vi "AlliGator Phasor Plot Panel.vi"() -> ()   [LabVIEW 2021, in "AlliGator Phasor Plot.lvlib"]
uses:
  AlliGator Phasor Plot.lvlib
  Phasor/Phasor (g, s).ctl
  Phasor/Phasor (m, phi).ctl
  AlliGator Phasor Plot Ctrl Refnums.ctl
  Globals, Variables, Constants/AlliGator Refnums List.ctl
  Utilities/Read-Write.ctl
  Settings/AlliGator Settings List.ctl
  Globals, Variables, Constants/AlliGator Variables List.ctl
  Palette/Image Palette Information.ctl
  Image/Image Display Palette Type.ctl
  Image/Image Display Event.ctl
  Image/Image Control Refnum.ctl
  <vilib>/Utility/miscctls.llb/LVPoint32TypeDef.ctl
  Action Engine/AlliGator Q Element.ctl
  Action Engine/AlliGator Q Event.ctl
  Image/Image Display User Event Data.ctl
  GUI/AlliGator Image Mouse Up Event Data.ctl
  Image/Image ROI Descriptor.ctl
  Image/Image Contour Definition.ctl
  Image/Image Contour ID.ctl
  Image/Image ROI Type.ctl
  Variant/Variant to Data/Variant to Boolean.vi
  Variant/Variant to Data/Variant to [String].vi
  Settings/AlliGator Settings+.lvlib
  Variant/Variant to Data/Variant to Data.lvlib
  Notebook/Notebook.lvlib
  Action Engine/AlliGator Action Engine.lvlib
  GUI/GUI.lvlib
  GUI/AlliGator GUI.lvlib
  Error/Error.lvlib
  Image/Image.lvlib
  Palette/Palette.lvlib
  Globals, Variables, Constants/AlliGator Globals, Variables & Constants.lvlib
  Python Plugins API/AlliGator Python Plugins.lvlib
  Phasor Graph/AlliGator Phasor Graph.lvlib
  Utilities/Utilities.lvlib
  Phasor/Phasor.lvlib
panel:
  out "True Phasor Plot Value":i32
  in  "Phasor ROI Decay":bool
  in  "Clear Phasor Overlay":bool
  in  "Highlight Phasor in Source Image":bool caption="Highlight Phasor ROI"
  in  "Image Overlay Color":u32(colorbox)=16777216
  in  "Overlay Mode":u16(ring)
  in  "Phasor Plot Active":bool
  in  "Pin Button":bool=TRUE
  in  "Phasor Plot ROI Color":u32(colorbox)=6618880
  in  "Refresh Phasor Plot":bool caption="Refresh Phsor Plot"
  out "Phasor Plot Image":T1(plugin-control)
  out "Phasor Plot Average Lifetime":dbl[unit]=nan caption="<tau>_a" format="%#_4e"
  out "Phasor Plot Phasor Ratio":dbl=nan caption="Amplitude Ratio (a1)" format="%#_4e"
  out "Phasor Plot Modulus Lifetime":dbl[unit]=nan caption="Modulus Lifetime" format="%#_4e"
  out "Phasor Plot Phase Lifetime":dbl[unit]=-9.431404035075279e-09 caption="Phase Lifetime" format="%#_4e"
  out "Phasor at cursor (m, phi)":T2={"m"=1.5330078000581284, "phi"=1.7786862539971595} caption="Phasor at Cursor (m, phi)" {"phi" format="%#_4e"; "m" format="%#_4e"}
  out "Phasor at cursor (g, s)":T3={"g"=-0.31640625, "s"=1.5} caption="Phasor at Cursor" {"s" format="%#.3e"; "g" format="%#_4e"}
  in  "Phasor Plot Color Scale":dbl(ramp)
  in  "Phasor Plot Display Range":cluster{u32, u32}(slide)={0, 100} scale=0.0..6578.0
  in  "Save Phasor Plot":bool
  out "Reference 2 Button":bool caption="Reference"
  out "Reference 1 Button":bool caption="Reference"
  in  "Phasor Plot Frequency":dbl[unit]=80000000.0 caption="Phasor Frequency"
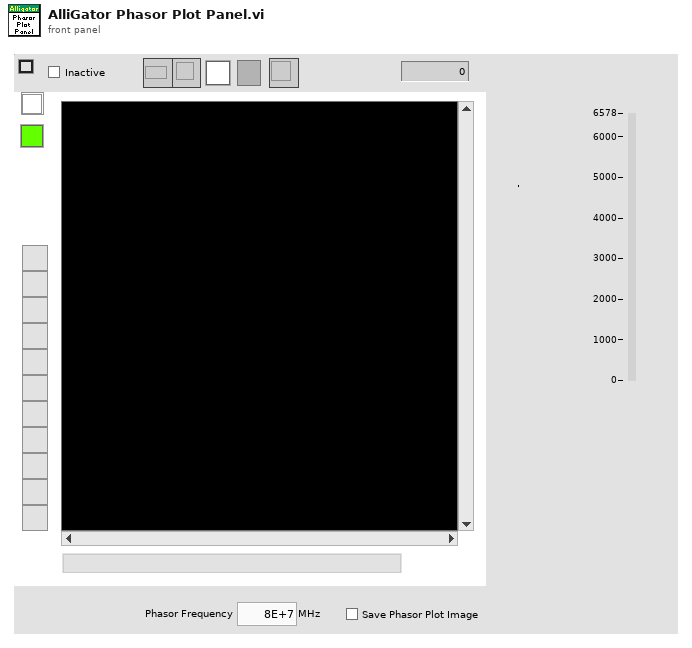
[diagram p1: front panel]
types:
  T1 = typedef "IMAQ Image.ctl" = refnum<image>
  T2 = typedef "Phasor.lvlib/Phasor (m, phi).ctl" = cluster{"m":dbl, "phi":dbl}
  T3 = typedef "Phasor.lvlib/Phasor (g, s).ctl" = cluster{"g":dbl, "s":dbl}
  T4 = typedef "Utilities.lvlib/Read-Write.ctl" = enum16{"Read", "Write"}
  T5 = typedef "AlliGator GUI.lvlib/AlliGator Refnums List.ctl" = enum16{"---------- AlliGator Control Refnums ----------", "AlliGator Tab Control Refnum", "Dataset Ctrl Refnums", "Image Histogram Ctrl Refnums", "Intensity Time Trace Ctrl Refnums", "Decay Graph Ctrl Refnums", "Decay Statistics Graph Ctrl Refnums", "Phasor Graph Ctrl Refnums", "Phasor Ratio Graph Ctrl Refnums", "Phasor Plot Ctrl Refnums", "Lifetime & Other Parameters Ctrl Refnums", "Decay Fit Parameter Map Ctrl Refnums", "Parameter Map Ctrl Refnums", "Other AlliGator Ctrl Refnums", "---------- AlliGator Menu Refnums ----------", "AlliGator Menu", "---------- IO Device ID ----------", "Mouse ID", "Keyboard ID"}
  T6 = typedef "AlliGator Phasor Plot.lvlib/AlliGator Phasor Plot Ctrl Refnums.ctl" = cluster{"Phasor Ratio":refnum<vi>, "Modulus Lifetime":refnum<vi>, "Phasor at cursor (m, phi)":refnum<vi>, "Phase Lifetime":refnum<vi>, "Phasor at cursor (g, s)":refnum<vi>, "Phasor Plor Average Lifetime":refnum<vi>, "Phasor Plot Active":refnum<vi>, "Save Phasor Plot":refnum<vi>, "Image Overlay Color":refnum<vi>, "Phasor Plot Color Scale":refnum<vi>, "Reference 1 Button":refnum<vi>, "Reference 2 Button":refnum<vi>, "True Phasor Plot Value":refnum<vi>, "Phasor Plot Display Range":refnum<vi>, "Phasor Plot Display":refnum<vi>, "Phasor Plot Frequency":refnum<vi>, "Overlay Mode":refnum<vi>}
  T7 = cluster{"Event Registration Refnum":refnum<event-registration>, "Phasor Plot Display Event":refnum<event-registration>, "Phasor Plote Display Range Event":refnum<event-registration>}
  T8 = typedef "AlliGator Settings+.lvlib/AlliGator Settings List.ctl" = enum16{"GUI:Visible Settings Tab", "GUI:Last Run Version", "Source Image:Use Image Histogram for Contrast", "Source Image:Low Count Pixels Rejection Options", "Source Image:High Count Pixels Rejection Options", "Source Image:Use Image Brightness", "Source Image:Blend Overlay with Image Background", "Source Image:Use Fixed ROI Diameter", "Source Image:ROI Diameter", "Source Image:ROI Center Color", "Source Image:Peak Threshold", "Source Image:Intensity Threshold", "Source Image:Image Binning Options", "Source Image:Image Smoothing Options", "Source Image:Image Histogram Active", "Source Image:Invert Binary Mask", "Source Image:Hot Pixel Removal", "Source Image:Overlay Analyzed ROI Center", "Source Image:Auto-Adjust Contrast", "Source Image:Histogram Lower Percentile", "Source Image:Histogram Upper Percentile", "Source Image:Lock ROI with Maps", "Source Image:Save Source Image", "Source Image:Scale Bar Options", "Source Image:Image Resolution (Pixel Size)", "Source Image:Flatfield Correction", "Source Image:Show Dead Left Columns Correction", "Source Image:Dead Left Columns Correction", "Source Image:Image Pre-Processing Operations Order", "Source Image:Overlay ROI Median", "Source Image:Median Overlay Color", "Data Information:Gate Width", "Data Information:Nanotime Gate Separation", "Data Information:Macrotime Gate Separation", "Data Information:Gate Step", "Data Information:# Gates", "Data Information:Gate Image Exposure", "Data Information:Gate Image Integration", "Data Information:Gates to Skip", "Data Information:Gates to Keep", "Data Information:Define Gates to", "Data Information:Channel Name", "Data Information:Available Channel Names", "Data Information:Channel Arithmetic", "Data Information:Background File Subtraction", "Data Information:Background File", "Data Information:Background Scaling Factor", "Data Information:Background Pile-up Correction", "Data Information:Background Pixel Well Capacity", "Data Information:Laser Period", "Data Information:SYNC Period", "Data Information:Pile-up Correction", "Data Information:Pixel Well Capacity", "Data Information:Dataset Scaling Factor", "Fluorescence Decay_Decay Pre-Processing:Reverse Gates", "Fluorescence Decay_Decay Pre-Processing:Verbose Decay Pre-Processing", "Fluorescence Decay_Decay Pre-Processing:Use Decay Pre-Processing", "Fluorescence Decay_Decay Pre-Processing:Background Subtraction", "Fluorescence Decay_Decay Pre-Processing:Background Definition Range", "Fluorescence Decay_Decay Pre-Processing:Baseline Subtraction Method", "Fluorescence Decay_Decay Pre-Processing:Decay Pre-Processing Operations Order", "Fluorescence Decay_Decay Pre-Processing:Smoothing Parameter", "Fluorescence Decay_Decay Pre-Processing:Shift Decay", "Fluorescence Decay_Decay Pre-Processing:Decay Shift Parameters", "Fluorescence Decay_Decay Pre-Processing:Fold Decay", "Fluorescence Decay_Decay Pre-Processing:# Folds", "Fluorescence Decay_Decay Pre-Processing:1-Normalize Decay", "Fluorescence Decay_Decay Pre-Processing:[0-1]-Normalize Decay", "Fluorescence Decay_Decay Pre-Processing:Smoothen Decay", "Fluorescence Decay_Decay Pre-Processing:Extrapolate Decay", "Fluorescence Decay_Decay Pre-Processing:Use Periodicity", "Fluorescence Decay_Decay Pre-Processing:Use Cursors", "Fluorescence Decay_Decay Pre-Processing:Tail Fraction", "Fluorescence Decay_Decay Pre-Processing:Head Fraction", "Fluorescence Decay_Decay Pre-Processing:Additional Points", "Fluorescence Decay_Decay Pre-Processing:Straighten Decay", "Fluorescence Decay_Decay Pre-Processing:Constant Background", "Fluorescence Decay_Decay Pre-Processing:Pixel-Normalize Decay", "Fluorescence Decay_Advanced Analysis:Extract IRF instead of Decay", "Fluorescence Decay_Advanced Analysis:IRF Extraction Options", "Fluorescence Decay_Advanced Analysis:IRF Optimization Options", "Fluorescence Decay_Advanced Analysis:Square Pulse Options", "Fluorescence Decay_Advanced Analysis:IRF Order", "Fluorescence Decay_Advanced Analysis:IRF Time Constants", "Fluorescence Decay_Advanced Analysis:Wavelet Analysis Options", "Fluorescence Decay_Advanced Analysis:Average Lifetime Options", "Fluorescence Decay_Fit Options:Fit Options", "Fluorescence Decay_Fit Options:Use Legacy Fitting Approach", "Fluorescence Decay_Fit Options:Use Data Information Laser Period", "Fluorescence Decay_Fit Parameters:Displayed Fit Parameters", "Fluorescence Decay_Fit Parameters:Fit Parameter Constraints", "Fluorescence Decay_Fit Parameters:Export Tabulated Results", "Fluorescence Decay_Fit Parameters:MLE Baseline Offset Type", "Fluorescence Decay_Fit Parameters:MLE Baseline Offset", "Fluorescence Decay_Fit Parameters:Guess Parameter Names", "Fluorescence Decay_Fit Parameters:Guess Parameter Values", "Fluorescence Decay_Fit Parameters:Guess Parameters Options", "Fluorescence Decay_Fit Parameters:Optimal Offset Selection Criterion", "Fluorescence Decay_Styles:Show Last Decay Only", "Fluorescence Decay_Styles:Decay Graph Color Array", "Fluorescence Decay:Decay Graph Active", "Fluorescence Decay Statistics:Min Peak Value", "Fluorescence Decay Statistics:Reject Low Decay Peak Pixels", "Fluorescence Decay Statistics:Reject High Decay Peak Pixels", "Fluorescence Decay Statistics:Max Peak Value", "Time Traces:Use File Timestamp", "Time Traces:Time Step", "Time Traces:Use Intensity Correction File", "Time Traces:Intensity Correction File", "Phasor Plot:Phasor Plot Smoothing Options", "Phasor Plot:Phasor Plot Size", "Phasor Plot:Phasor Plot Graphics Options", "Phasor Plot:Cumulative Phasor Plot", "Phasor Plot:Use Phasor Brightness", "Phasor Plot:Blend Overlay with Phasor Background", "Phasor Plot:Save Phasor Plot", "Phasor Plot:Show References", "Phasor Plot:Phasor Ratio Decay Range", "Phasor Plot:Exponential Fading", "Phasor Plot:Phasor Ratio Reference Colors", "Phasor Plot:Reference Radius", "Phasor Plot:Show Color Map Vertices", "Phasor Plot:Phasor Plot Active", "Phasor Plot:Phasor Ratio Color Map Type", "Phasor Plot:Phasor Ratio Color Map", "Phasor Plot:Phasor Ratio Display Range", "Phasor Plot:Selected Image ROI(s)", "Phasor Plot:All Image ROIs", "Phasor Plot:Selected Phasor Plot ROI(s)", "Phasor Plot:All Phasor Plot ROIs", "Phasor Plot:Phasor Ratio Color-Coded Quantity", "Phasor Plot:Store Phasor Harmonics", "Phasor Plot:Draw Reference Segment", "Phasor Plot:User-Defined Quantity", "Phasor Plot:Color Scale High Color", "Phasor Plot:Color Scale Low Color", "Phasor Plot:Intensity-weighted Phasor Plot", "Phasor Graph:Phasor Frequency", "Phasor Graph:Phasor Ratio Type", "Phasor Graph:Pixel-level Phasor Computation", "Phasor Graph:Save Phasor Graph", "Phasor Graph:Phasor Graph Active", "Phasor Graph:Phasor SDV Options", "Phasor Graph:Intensity-weighted Phasor Graph", "Phasor Graph:Define Shortest Lifetime as", "Phasor Calibration:Use Backup Calibration if needed", "Phasor Calibration:Backup Calibration Type", "Phasor Calibration:Calibration Type", "Phasor Calibration:Calibration Lifetime", "Phasor Calibration:Calibration Map Algorithm", "Single-Exponential Phasor Locus (SEPL):Gate Parameters", "Single-Exponential Phasor Locus (SEPL):User-defined Gate", "Single-Exponential Phasor Locus (SEPL):User-defined IRF", "Single-Exponential Phasor Locus (SEPL):Phasor Parameters", "Single-Exponential Phasor Locus (SEPL):Decay & IRF Parameters", "Single-Exponential Phasor Locus (SEPL):Display Parameters", "Lifetime Analysis:Decay Analysis Parameters", "Lifetime Analysis:Lifetime Map Active", "Plugins:Python Settings", "Miscellaneous:Verbose Mode", "Miscellaneous:Beep after Script", "Miscellaneous:Saved Image File Format", "Miscellaneous:Exported Gate Image Settings", "Miscellaneous:Include Loading in Timing", "Miscellaneous:Verbose Settings Mode", "Miscellaneous:Histogram Options", "Miscellaneous:Beep on Error", "Miscellaneous:# Logical Processors Used", "Miscellaneous:ROI Description Max Characters", "Miscellaneous:Verbose Error Mode", "Miscellaneous:Transparent Mask Color"}
  T9 = typedef "Palette.lvlib/Image Palette Information.ctl" = cluster{"Palette Name [# Colors,int?,inv?]":string, "Palette Type":T10, "Palette Colors":u32[], "Interpolate?":bool}
  T10 = typedef "Image.lvlib/Image Display Palette Type.ctl" = u32
  T11 = typedef "AlliGator Globals, Variables & Constants.lvlib/AlliGator Variables List.ctl" = enum16{"---- GUI ----", "GUI:Initialization Status", "GUI:State Indicators Refnum", "GUI:Original AlliGator Menu Items", "GUI:Current Action Loop State", "GUI:Script in progress", "GUI:Playback", "GUI:Loop Playback", "GUI:Search ROI Used", "GUI:Search ROI", "Image Histogram Max Legend Size", "Decay Graph Max Legend Size", "Intensity Graph Max Legend Size", "Decay Statistics Graph Max Legend Size", "Phasor Graph Max Legend Size", "Phasor Ratio Graph Max Legend Size", "Lifetime Graph Max Legend Size", "---- Files ----", "Files:Export Dataset Frames as Individual Files", "Files:Show Batch Export Help Balloons", "Files:Frames in Dataset", "Files:ptu File Frame Start Indices", "Files:Current Frame in Dataset", "Files:Current Frame Timestamp", "Files:Dataset Loaded", "Files:Dataset Metadata", "Files:Dataset Channel", "Files:Dataset Data Description", "Files:Background Dataset Metadata", "Files:Background Dataset Channel", "Files:Background Dataset Data Description", "Files:Background File Subtraction", "Files:Background File Path", "Files:Background File Pile-up Correction", "Files:Background File Pixel Well Capacity", "Files:Background File Scaling Factor", "Files:Current Dataset Load Settings", "Files:Dataset Path", "Files:ICCD-specific Information", "Files:Macrotime Gate Separation", "------ Python Plugins ------", "Python Plugins:Information", "Python Plugins:Python Session", "Python Plugins:Valid Python Session?", "---- Source Image ----", "Source Image:ROIs", "Source Image:Current ROI", "Source Image:ROI Event Refnum", "X_Source Image:Display Range", "X_Source Image:Palette Information", "X_Source Image:Type of Displayed Image", "X_Time Gate Slider", "Source Image:Palette List", "Source Image:Scale", "Source Image:ROI Overlay Color", "Source Image:Overlay to Erase", "Source Image:Is Displayed Image Accumulated", "Source Image:White Light Image Modified", "Source Image:Mask Image Modified", "---- Image Profile Window ----", "Image Profile:Window Event Refnum", "Image Profile:IntensityType", "Image Profile:Intensity Average Type", "Image Profile:Intensity-weighted SDV", "Image Profile:Box Profile Type", "Image Profile:Window Open", "Image Profile:Plotted Fit Parameter", "------ Phasor Graph -------", "Phasor Graph:Show Line", "---- Phasor Plot ---", "Phasor Plot:Parameters Changed", "Phasor Plot:FLI Dataset Modified since last Calculation", "Phasor Harmonics Data", "Selected Phasor Harmonics", "Phasor Harmonic Manager Event Refnum", "Phasor Plot:ROIs", "Phasor Plot:Current ROI", "Phasor Plot:ROI Event Refnum", "Phasor Plot:Image Reference Points", "Phasor Plot:Computed", "Phasor Plot:Palette Information", "Phasor Plot:Palette List", "Phasor Plot:Phasor Ratio Palette Information", "Phasor Plot:Phasor Ratio Palette List", "Phasor Plot:Image Scale", "Phasor Plot:Image Overlay to Erase", "Phasor Plot:Image Elements to Update", "Phasor Plot:Current Calculation Parameters", "Phasor Plot:Current Calibration Options", "Phasor Plot:Reset Cumulated Phasor Plot", "Phasor Plot:Reference 1", "Phasor Plot:Lifetime Reference 1", "Phasor Plot:Reference 1 Frequency", "Phasor Plot:Reference 2", "Phasor Plot:Lifetime Reference 2", "Phasor Plot:Reference 2 Frequency", "---- Decay Analysis ----", "Number of Selected Decays to Fit", "LS Fit Results", "LAR Fit Results", "BS Fit Results", "Last Decay Max - Min", "Best Fit Parameters", "Best Fit Parameter Names", "Actual Size X", "Actual Size Y", "Binning X", "Binning Y", "Actual # Gates", "Dataset Number", "Gates to...", "Gates Skipped", "Gates to keep", "Gate Step", "Gate Separation", "Reversed Gates", "Pile-up Correction", "Pixel Well Capacity", "Background Subtracted", "Background Subtraction Method", "Background Definition Range", "Background File (deprecated)", "Number of Dataset Accumulated", "Array of Accumulated Dataset Paths", "Do Averaged Datasets", "Destination File Path", "Process Plot Target", "Use 1/D as Phasor Frequency", "---- Decay Fit Parameter Map -----", "Decay Fit Parameter Map:Palette Information", "Decay Fit Parameter Map:Palette List", "Decay Fit Parameter Map:X Resolution", "Decay Fit Parameter Map:Y Resolution", "Decay Fit Parameter Map:Use Decay Fit Result Constraints", "Decay Fit Parameter Map:Decay Fit Result Constraints", "Decay Fit Parameter Map:Decay Fit Result Constraints Applied", "---- Parameter Map ----", "Parameter Map:Palette Information", "Parameter Map:Palette List", "------- Local Decay Window ---------", "Local Decay Graph Window:Event Refnum", "Local Decay Graph Window:Use normalized IRF for convolution", "----- Miscellaneous ----", "Misc:Skippable Dialog Windows Status"}
  T12 = enum16{"0", "1", "2", "3", "4", "5", "6", "7", "8", "9", "A", "B", "C", "D", "E", "F", "G", "H", "I", "J", "K", "L", "M", "N", "O", "P", "Q", "R", "S", "T", "U", "V", "W", "X", "Y", "Z", "F1", "F2", "F3", "F4", "F5", "F6", "F7", "F8", "F9", "F10", "F11", "F12", "F13", "F14", "F15", "ADD", "BACK", "BACKSLASH", "CAPITAL", "COMMA", "DECIMAL", "DELETE", "DIVIDE", "DOWN", "END", "EQUALS", "ESCAPE", "GRAVE (`)", "HOME", "INSERT", "LBRACKET", "LCONTROL", "LEFT", "L ALT", "LSHIFT", "LWIN", "MINUS", "MULTIPLY", "NEXT", "NUMLOCK", "NUMPAD_0", "NUMPAD_1", "NUMPAD_2", "NUMPAD_3", "NUMPAD_4", "NUMPAD_5", "NUMPAD_6", "NUMPAD_7", "NUMPAD_8", "NUMPAD_9", "PAUSE", "PERIOD", "PRIOR (PG UP)", "RBRACKET", "RCONTROL", "RETURN", "RIGHT", "R ALT", "RSHIFT", "RWIN", "SCROLL", "SEMICOLON", "SLASH", "SPACE", "SUBTRACT", "TAB", "UP", "ENTER (num pad)", "' (quote)"}
  T13 = typedef "Image.lvlib/Image Display Event.ctl" = cluster{"Item Tag":string, "Image Control Refnum":T14, "Coords":T15, "Item Path":string}
  T14 = typedef "Image.lvlib/Image Control Refnum.ctl" = refnum<vi>
  T15 = typedef "LVPoint32TypeDef.ctl" = cluster{"Horizontal":i32, "Vertical":i32}
  T16 = typedef "AlliGator Action Engine.lvlib/AlliGator Q Element.ctl" = cluster{"AlliGator Q Event":T17, "Data":variant}
  T17 = typedef "AlliGator Action Engine.lvlib/AlliGator Q Event.ctl" = enum16{"---- Files ----", "Files:Set Batch Export Files To Save", "Files:Set Dataset Loading & Pre-processing Options", "Files:Check #Frames in Dataset", "Files:Increment Frame Index", "Files:Open Mask Image", "Files:Open White Light Image", "Files:Open Single Dataset", "Files:New Folder of Folders Selected", "Files:Load File (all Types)_Scriptable", "Files:Move Flattened Series to Folders Series", "Files:Select Folder", "Files:Load FLI Dataset", "Files:Load Swiss SPAD 1 Dataset", "Files:Load Swiss SPAD 2 Dataset", "Files:Load .sdt FLI Dataset", "Files:Load .ptu FLI Dataset", "Files:Load .bin FLI Dataset", "Files:Load Single Gate Image Folder", "Files:Load I/m/phi Dataset (deprecated)", "Files:Load Single Image", "Files:Subtract Background File", "Files:Export FLI Dataset", "Files:Load HDF5 FLI Dataset", "Files:Set Destination File Path", "Files:Save Mask Image", "Files:Batch Conversion", "Files:New Folder Selected", "Files:Close FLI Dataset", "Files:Close FLI Dataset Series", "Files:Close White Light Image", "Files:Close Mask Image", "---- FLI Dataset ----", "FLI Dataset:Channel Arithmetic", "FLI Dataset:Export Average Lifetime Map as ASCII", "FLI Dataset:Export User-Defined Quantity Map as ASCII", "FLI Dataset:Python Function FLI Dataset Event", "FLI Dataset:ROI Analysis", "FLI Dataset:Tilted Logistic Square Gated IRF Characteristics Map", "FLI Dataset:Logistic Square Gated IRF Characteristics Map", "FLI Dataset:Square Gated IRF Characteristics Map", "FLI Dataset:Multi-ROI Single-Pixel Phasor Analysis", "FLI Dataset:Multi-ROI Single-Pixel NLSF Analysis", "FLI Dataset:All ROIs IRF Extraction", "FLI Dataset:All ROIs Decay Fit Non-Interactive (Fast + Individual IRF)", "FLI Dataset:All ROIs Phasor Analysis", "FLI Dataset:All ROIs Decay Fit", "FLI Dataset:Fluorescence Decay Statistics", "FLI Dataset:Update Decay Statistics Graph", "FLI Dataset:Get Decay from ROI", "FLI Dataset:All ROIs Average Lifetimes", "FLI Dataset:Save/Load Local IRFs", "FLI Dataset:Clear Local IRFs", "FLI Dataset:Phasor Calibration Maps (# Gates Series) Script", "FLI Dataset:Calibrated Phasor Map Series", "---- FLI Dataset Series ----", "FLI Dataset Series:Sum All Datasets in Series", "FLI Dataset Series:Add Dataset to Accumulated Dataset", "FLI Dataset Series:Display Accumulated Dataset", "FLI Dataset Series:Clear Dataset Series Sum", "FLI Dataset Series:Time-Series Analysis (NLSF)", "FLI Dataset Series:Time-Series Analysis (Phasor)", "---- Image ----", "Image:Update Image Profile Plots", "Image:Image Histogram Cursor Move", "Image:Image Histogram", "Image:Image Contrast", "Image:Set Image Histogram Cursor Move Flag", "Image:Clear Image Overlay", "Image:Use ROI as Search Area", "Image:Set ROI Diameter", "Image:Save Image Data as TIFF", "Image:Save Displayed Image with Overlay", "Image:Save Image Overlay Only", "Image:Save Image as Hot Pixel Mask", "Image:Change Source Image Color Palette", "Image:Copy Image to Clipboard", "Image:Source Image ROI Selection", "Image:Delete All ROIs", "Image:Delete All Unselected ROIs", "Image:Delete ROI", "Image:Merge All ROIs", "Image:Store ROI", "Image:Source Image ROI Storage", "Image:Export ROI Description to Notebook", "Image:Save ROI", "Image:Load ROI", "Image:Paste ROI Definition", "Image:Clear ROI", "Image:Identify ROIs in Mask Image", "Image:Create Complementary ROI", "Image:Create Contour ROI", "Image:Create ROI(s) from Pixels with Peak above Min_Scriptable", "Image:Create ROI(s) from Pixels with Intensity above Min_Scriptable", "Image:Compute ROI Statistics", "Image:Delete ROI(s) based on ROI Characteristics", "Image:Create ROI Grid", "Image:ROI to Individual Pixel ROIs", "Image:Python Function Source Image Event", "Image:Show Phasor Calibration Map ROI Centers", "Image:Convert ROI to Mask Image", "Image:Mouse Move", "Image:Mouse Up", "Image:Set Source Image Mouse Move Flag", "Image:Add Scale Bar Overlay", "Image:Delete Existing ROIs Option", "Image:Overlay ROI Median", "Image:Check Current ROI", "Image:Update True Pixel Value", "Image:Use ROI", "---- Decay ----", "Decay:Clear IRF/Reference Plot", "Decay:Add Decay to Graph", "Decay:Smoothen Plot", "Decay:Smoothen Plot Tail", "Decay:Average Selected Plots", "Decay:Extract IRF", "Decay:Optimal IRF Extraction", "Decay:Threshold IRF", "Decay:Fit to Model IRF", "Decay:Fit IRF to Square Gate", "Decay:Fit IRF to Logistic Square Gate", "Decay:Fit IRF to Tilted Logistic Square Gate", "Decay:Create Bounding Cursors Set", "Decay:Export Bounding Cursors Definition to Notebook", "Decay:Denoise Plot", "Decay:Compute Cumulative Function", "Decay:Use as Reference Decay", "Decay:Show Reference Decay/IRF", "Decay:Extrapolate Decay", "Decay:Create Head & Tail Bounding Cursors", "Decay:Store Cursor-defined Head & Tail Fractions", "Decay:Rebin Plot", "Decay:1-Normalize Decay", "Decay:[0-1]-Normalize Plot", "Decay:Straighten Decay", "Decay:Shift Decay", "Decay:Fold Decay", "Decay:Fit Decay", "Decay:Global Fit of Selected Decays", "Decay:Post Global Fit Script", "Decay:Add Global Fit Parameters to Graph", "Decay:Add Decay Parameter(s) to Plot (Graph)", "Decay:Export Decay to Phasor Graph", "Decay:Compute Average Lifetime", "Decay:Plot Convolution", "Decay:Graph Tip Strip Update", "---- Decay Statistics ----", "Decay Statistics:Tip Strip Update", "---- Intensity Time Trace ----", "Intensity Time Trace:Use File Timestamp", "Intensity Time Trace:Load Intensity Corrections File", "Intensity Time Trace:Clear Intensity Corrections File", "Intensity Time Trace:Tip Strip Update", "---- Phasor Plot ----", "Phasor Plot:Build Phasor Plot", "Phasor Plot:Change Phasor Plot Color Palette", "Phasor Plot:Adjust Phasor Plot Display Range", "Phasor Plot:Highlight Image ROI in Phasor Plot", "Phasor Plot:Save Phasor Plot Image with Overlay", "Phasor Plot:Export Complex Phasor Map", "Phasor Plot:Export Phasor Ratio Map", "Phasor Plot:Export Average Lifetime Map", "Phasor Plot:Compute Phase Lifetime Histogram", "Phasor Plot:Compute Phasor Ratio Histogram", "Phasor Plot:Compute Phase Lifetime vs Intensity Scatter Plot", "Phasor Plot:Weber 2-Component Decomposition", "Phasor Plot:Update Phasor Color Map Vertices", "Phasor Plot:Clear Phasor Overlay", "Phasor Plot:Use Segment Extremities as References", "Phasor Plot:Use UC/Segment Intersections as References", "Phasor Plot:Use UC/Principal Axis Intersections as References", "Phasor Plot:Use UC/Linear Fit Intersections as References", "Phasor Plot:Update Phasor Plot Reference", "Phasor Plot:Show Local Phasor Info in Phasor Plot", "Phasor Plot:Update Phasor Plot State", "Phasor Plot:Phasor Plot ROI Storage", "Phasor Plot:Phasor Plot ROI Selection", "Phasor Plot:Python Function Phasor Plot Event", "Phasor Plot:Overlay Phasor ROI, Ratio or Map in Source Image", "Phasor Plot:Compute Decay of Selected Phasors", "Phasor Plot:Phasor at Image Pixel", "Phasor Plot:Mouse Move", "Phasor Plot:Mouse Up", "Phasor Plot:Display Range Mouse Move", "Phasor Plot:Set Mouse Move Flag", "Phasor Plot:Update True Phasor Plot Value", "---- Phasor Graph ----", "Phasor Graph:Get Phasor Value", "Phasor Graph:Create New Phasor Plot Dialog", "Phasor Graph:Update Last Phasor Value", "Phasor Graph:Update Phasor (m, phi)", "Phasor Graph:Remove Single Phasor from Plot", "Phasor Graph:Add Single Phasor to Plot", "Phasor Graph:Remove Phasor Plot", "Phasor Graph:Remove Selected Phasor Plots", "Phasor Graph:Clear Phasor Data", "Phasor Graph:Clear Phasor Graph", "Phasor Graph:Cursor Move", "Phasor Graph:Draw Cursor Connecting Line", "Phasor Graph:Clear Cursor Connecting Line", "Phasor Graph:Find UC Intersection", "Phasor Graph:Use UC/Cursor-Defined Line Intersections", "Phasor Graph:Use Selected Plots Fitted Line/UC Intersections", "Phasor Graph:Use Selected Plots Principal Axis/UC Intersections", "Phasor Graph:Show Single Phasor", "Phasor Graph:Save Single Phasor Plot", "Phasor Graph:Save All Phasor Plots", "Phasor Graph:Load Phasor Plot(s)", "Phasor Graph:Phasor Multiplication", "Phasor Graph:Compute Average Phasor", "Phasor Graph:Compute Multiple Average Phasors (Selected Plots)", "Phasor Graph:Export Single Phasor Plot Phase Lifetimes", "Phasor Graph:Parameter 2 vs Parameter 1 Scatter Plot", "Phasor Graph:Use Cursor n Location", "Phasor Graph:Set Reference n to Current Phase Lifetime Value", "Phasor Graph:Set Reference n to Lifetime Value", "Phasor Graph:Set Cursor n Location", "Phasor Graph:Save Phasor Graph Image", "Phasor Graph:Update SEPL Plot", "Phasor Graph:Export Single Phasor Plot Data", "Phasor Graph:Export Selected Phasor Plots Data", "Phasor Graph:Python Function Phasor Graph Event", "Phasor Graph:Tip Strip Update", "---- Calibration ----", "Calibration:Set Calibration Type", "Calibration:Load/Save Phasor Calibration", "Calibration:Load/Save Phasor Calibration Series", "Calibration:Load/Save Phasor Calibration Map", "Calibration:Use as Calibration", "Calibration:Compute Optimal Calibration from Phasor References", "Calibration:Clear Phasor Calibration", "Calibration:Single Phasor Calibration Information", "Calibration:Use as Calibration Series", "Calibration:Use as Calibration Map", "Calibration:Clear Calibration Series", "Calibration:Phasor Calibration Series Information", "Calibration:Clear Calibration Map", "Calibration:Phasor Calibration Map Information", "Calibration:Apply Phasor Calibration", "Calibration:Update Single Plot Calibration", "Calibration:Update Multiple Plots Calibration", "Calibration:Clear Single Plot Calibration", "Calibration:Clear All Plots Calibrations", "Calibration:Clear Plot(s) Calibration(s)?", "---- Phasor Ratio ----", "Phasor Ratio:Clear Reference n", "Phasor Ratio:Toggle Selected Plot(s)  Lock to Reference 1", "Phasor Ratio:Use as Reference n", "Phasor Ratio:Send Reference n to Notebook", "Phasor Ratio:Toggle Selected Plot(s)  Lock to Reference 2", "Phasor Ratio:Compute Phasor Ratio at Mouse Location", "Phasor Ratio:Compute Phasor Plot's Average Phasor Ratio", "Phasor Ratio:Compute Time-Series Phasor Ratios", "Phasor Ratio:Fit Line to Phasor Ratio Plot", "Phasor Ratio:Save References", "Phasor Ratio:Load References", "Phasor Ratio:Update Phasor Reference 1", "Phasor Ratio:Update Phasor Reference 2", "Phasor Ratio:Move Cursor n to Reference n", "Phasor Ratio:Use as Phasor Reference 1 Lifetime", "Phasor Ratio:Use as Phasor Reference 2 Lifetime", "Phasor Ratio:Export Phasor Ratio Map as ASCII", "Phasor Ratio:Tip Strip Update", "---- Lifetime & Other Parameters Graph ----", "Lifetime:Compute Sliced Mean, SDV and CV Plots", "Lifetime:Plot Decay Shifts", "Lifetime:Plot Histogram", "---- Decay Fit Parameter Map ----", "Decay Fit Parameter Map:Export ROI NLSF Data as ASCII", "Decay Fit Parameter Map:Set Decay Fit Parameter Map Selection", "Decay Fit Parameter Map:Build Decay Fit Parameter Map", "Decay Fit Parameter Map:Change Decay Fit Parameter Map Color Palette", "Decay Fit Parameter Map:Export Decay Fit Parameter Map Data as ASCII", "Decay Fit Parameter Map:Export All Decay Fit Parameter Maps Data as ASCII", "Decay Fit Parameter Map:Selected Parameter Scatterplot", "Decay Fit Parameter Map:Parameter 2 vs Parameter 1 Scatterplot", "Decay Fit Parameter Map:Save Decay Fit Parameter Map Image", "Decay Fit Parameter Map:Save-Load IRFs & Fit Data", "Decay Fit Parameter Map:Update Local Decay Plots", "Decay Fit Parameter Map:Python Function Decay Fit Parameters Map Event", "Decay Fit Parameter Map:Overlay Decay Fit Parameter Map in Source Image", "Decay Fit Parameter Map:Selected Parameter vs Intensity Scatterplot", "Decay Fit Parameter Map:Mouse Up", "Decay Fit Parameter Map:Mouse Move", "Decay Fit Parameter Map:Display Range Mouse Move", "Decay Fit Parameter Map:Change Map Resolution", "Decay Fit Parameter Map:Variance Significance Maps", "Decay Fit Parameter Map:Fit Result Constraints Window", "Decay Fit Parameter Map:Use ROI", "---- Parameter Map ----", "Parameter Map:Export ROI Parameters Data as ASCII", "Parameter Map:Add Parameter Map Set", "Parameter Map:Delete Parameter Map Set", "Parameter Map:Update Parameter List", "Parameter Map:Build Parameter Map", "Parameter Map:Change Parameter Map Color Palette", "Parameter Map:Export Parameter Map Data as ASCII", "Parameter Map:Export All Parameter Maps Data as ASCII", "Parameter Map:Selected Parameter Scatterplot", "Parameter Map:Parameter 2 vs Parameter 1 Scatterplot", "Parameter Map:Selected Parameter vs Intensity Scatterplot", "Parameter Map:Save Parameter Map Image", "Parameter Map:Save-Load IRFs & Parameter Maps (TODO)", "Parameter Map:Set Parameter Map Selection", "Parameter Map:Python Function Parameter Map Event", "Parameter Map:Overlay Parameter Map in Source Image", "Parameter Map:Update Local Decay Plots", "Parameter Map:Mouse Up", "Parameter Map:Mouse Move", "Parameter Map:Display Range Mouse Move", "Parameter Map:Use ROI", "---- Generic Graph ----", "Generic Graph:Generic XY Graph Event", "Generic Graph:Python Function XY Graph Event", "Generic Graph:New Plot", "Generic Graph:Save Plot", "Generic Graph:XY Plot Histogram", "Generic Graph:Set XY Graph Plot Name", "Generic Graph:Set Last Cursor Style", "Generic Graph:Tip Strip Update", "---- GUI ----", "GUI:Start Script", "GUI:Type of Displayed Image Changed", "GUI:Gate Image Slide Changed", "GUI:Show Busy Icon", "GUI:Show Busy Icon & Abort Button", "GUI:Hide Busy Icon", "GUI:Hide Busy Icon & Abort Button", "GUI:Abort", "GUI:End Script", "GUI:Start Timing", "GUI:End Timing", "GUI:Set State Indicator", "GUI:Send Parameters JSON Strings to Clipboard", "GUI:Set Gate Step", "GUI:Idle", "GUI:Initialization", "GUI:Quit", "GUI:Increment Dataset Index", "GUI:Set Dataset Index to -1", "GUI:Time Series Slider Moved", "GUI:Time Series Slider Changed", "GUI:Toggle Playback or Loop", "GUI:Playback Script", "GUI:Set Phasor Frequency", "GUI:Open Window", "GUI:Start Test Script", "GUI:End Test Script", "GUI:Set Verbose Mode", "GUI:Set Verbose Settings Mode", "GUI:Initialize Python Session", "DEBUG"}
  T18 = typedef "Image.lvlib/Image Display User Event Data.ctl" = cluster{"Image Control Refnum":T14, "Coords":T15, "button info":cluster{"button 1":bool, "button 2":bool, "button 3":bool, "button 4":bool}, "keys pressed":enum16{"0", "1", "2", "3", "4", "5", "6", "7", "8", "9", "A", "B", "C", "D", "E", "F", "G", "H", "I", "J", "K", "L", "M", "N", "O", "P", "Q", "R", "S", "T", "U", "V", "W", "X", "Y", "Z", "F1", "F2", "F3", "F4", "F5", "F6", "F7", "F8", "F9", "F10", "F11", "F12", "F13", "F14", "F15", "ADD", "BACK", "BACKSLASH", "CAPITAL", "COMMA", "DECIMAL", "DELETE", "DIVIDE", "DOWN", "END", "EQUALS", "ESCAPE", "GRAVE (`)", "HOME", "INSERT", "LBRACKET", "LCONTROL", "LEFT", "L ALT", "LSHIFT", "LWIN", "MINUS", "MULTIPLY", "NEXT", "NUMLOCK", "NUMPAD_0", "NUMPAD_1", "NUMPAD_2", "NUMPAD_3", "NUMPAD_4", "NUMPAD_5", "NUMPAD_6", "NUMPAD_7", "NUMPAD_8", "NUMPAD_9", "PAUSE", "PERIOD", "PRIOR (PG UP)", "RBRACKET", "RCONTROL", "RETURN", "RIGHT", "R ALT", "RSHIFT", "RWIN", "SCROLL", "SEMICOLON", "SLASH", "SPACE", "SUBTRACT", "TAB", "UP", "ENTER (num pad)", "' (quote)"}[]}
  T19 = typedef "AlliGator GUI.lvlib/AlliGator Image Mouse Up Event Data.ctl" = cluster{"Current ROI Tool":u32, "ROI Descriptor":T20, "Shift":bool, "Alt":bool, "Image Display Refnum":T14}
  T20 = typedef "Image.lvlib/Image ROI Descriptor.ctl" = cluster{"Global Rectangle":i32[], "Contours":T21[]}
  T21 = typedef "Image.lvlib/Image Contour Definition.ctl" = cluster{"Contour Type":T22, "ROI Type":T23, "Points":i32[]}
  T22 = typedef "Image.lvlib/Image Contour ID.ctl" = enum32{"External", "Internal"}
  T23 = typedef "Image.lvlib/Image ROI Type.ctl" = enum16{"No Selection", "Point", "Line", "Rectangle", "Oval", "Polygon", "Freehand Region", "Annulus", "Unused2", "Unused3", "Broken Line", "Freehand Line", "Rotated Rectangle"}
  T24 = enum16{"0", "1", "2", "3", "4", "5", "6", "7", "8", "9", "A", "B", "C", "D", "E", "F", "G", "H", "I", "J", "K", "L", "M", "N", "O", "P", "Q", "R", "S", "T", "U", "V", "W", "X", "Y", "Z", "F1", "F2", "F3", "F4", "F5", "F6", "F7", "F8", "F9", "F10", "F11", "F12", "F13", "F14", "F15", "ADD", "BACK", "BACKSLASH", "CAPITAL", "COMMA", "DECIMAL", "DELETE", "DIVIDE", "DOWN", "END", "EQUALS", "ESCAPE", "GRAVE (`)", "HOME", "INSERT", "LBRACKET", "LCONTROL", "LEFT", "L ALT", "LSHIFT", "LWIN", "MINUS", "MULTIPLY", "NEXT", "NUMLOCK", "NUMPAD_0", "NUMPAD_1", "NUMPAD_2", "NUMPAD_3", "NUMPAD_4", "NUMPAD_5", "NUMPAD_6", "NUMPAD_7", "NUMPAD_8", "NUMPAD_9", "PAUSE", "PERIOD", "PRIOR (PG UP)", "RBRACKET", "RCONTROL", "RETURN", "RIGHT", "R ALT", "RSHIFT", "RWIN", "SCROLL", "SEMICOLON", "SLASH", "SPACE", "SUBTRACT", "TAB", "UP", "ENTER (num pad)", "' (quote)"}[]
  T25 = typedef "AlliGator Phasor Graph.lvlib/AlliGator Phasor Graph Ctrl Refnums.ctl" = cluster{"Phasor Ratio":refnum<vi>, "Modulus Lifetime":refnum<vi>, "Phasor at cursor (m, phi)":refnum<vi>, "Phase Lifetime":refnum<vi>, "Phasor at cursor (g, s)":refnum<vi>, "Phasor Graph Average Lifetime":refnum<vi>, "Phasor Graph Active":refnum<vi>, "Save Phasor Graph":refnum<vi>, "Phasor Frame Slide":refnum<vi>, "Single Step Phasor":refnum<vi>, "Calibration Type":refnum<vi>, "Show Line":refnum<vi>, "Phase Lifetime 1":refnum<vi>, "Phase Lifetime 2":refnum<vi>, "Phasor Graph Frequency":refnum<vi>, "Phasor Reference 1 Control":refnum<vi>, "Phasor Reference 2 Control":refnum<vi>, "Calibration Lifetime":refnum<vi>, "Phase Lifetime SDV":refnum<vi>, "Average Lifetime SDV":refnum<vi>, "Phasor Ratio SDV":refnum<vi>, "Modulus Lifetime SDV":refnum<vi>, "Phasor Graph":refnum<vi>}
  T26 = cluster{"button 1":bool, "button 2":bool, "button 3":bool, "button 4":bool}
  T27 = cluster{"Global Rectangle":i32[], "Contours":cluster{"Contour Type":u32, "ROI Type":u32, "Points":i32[]}[]}
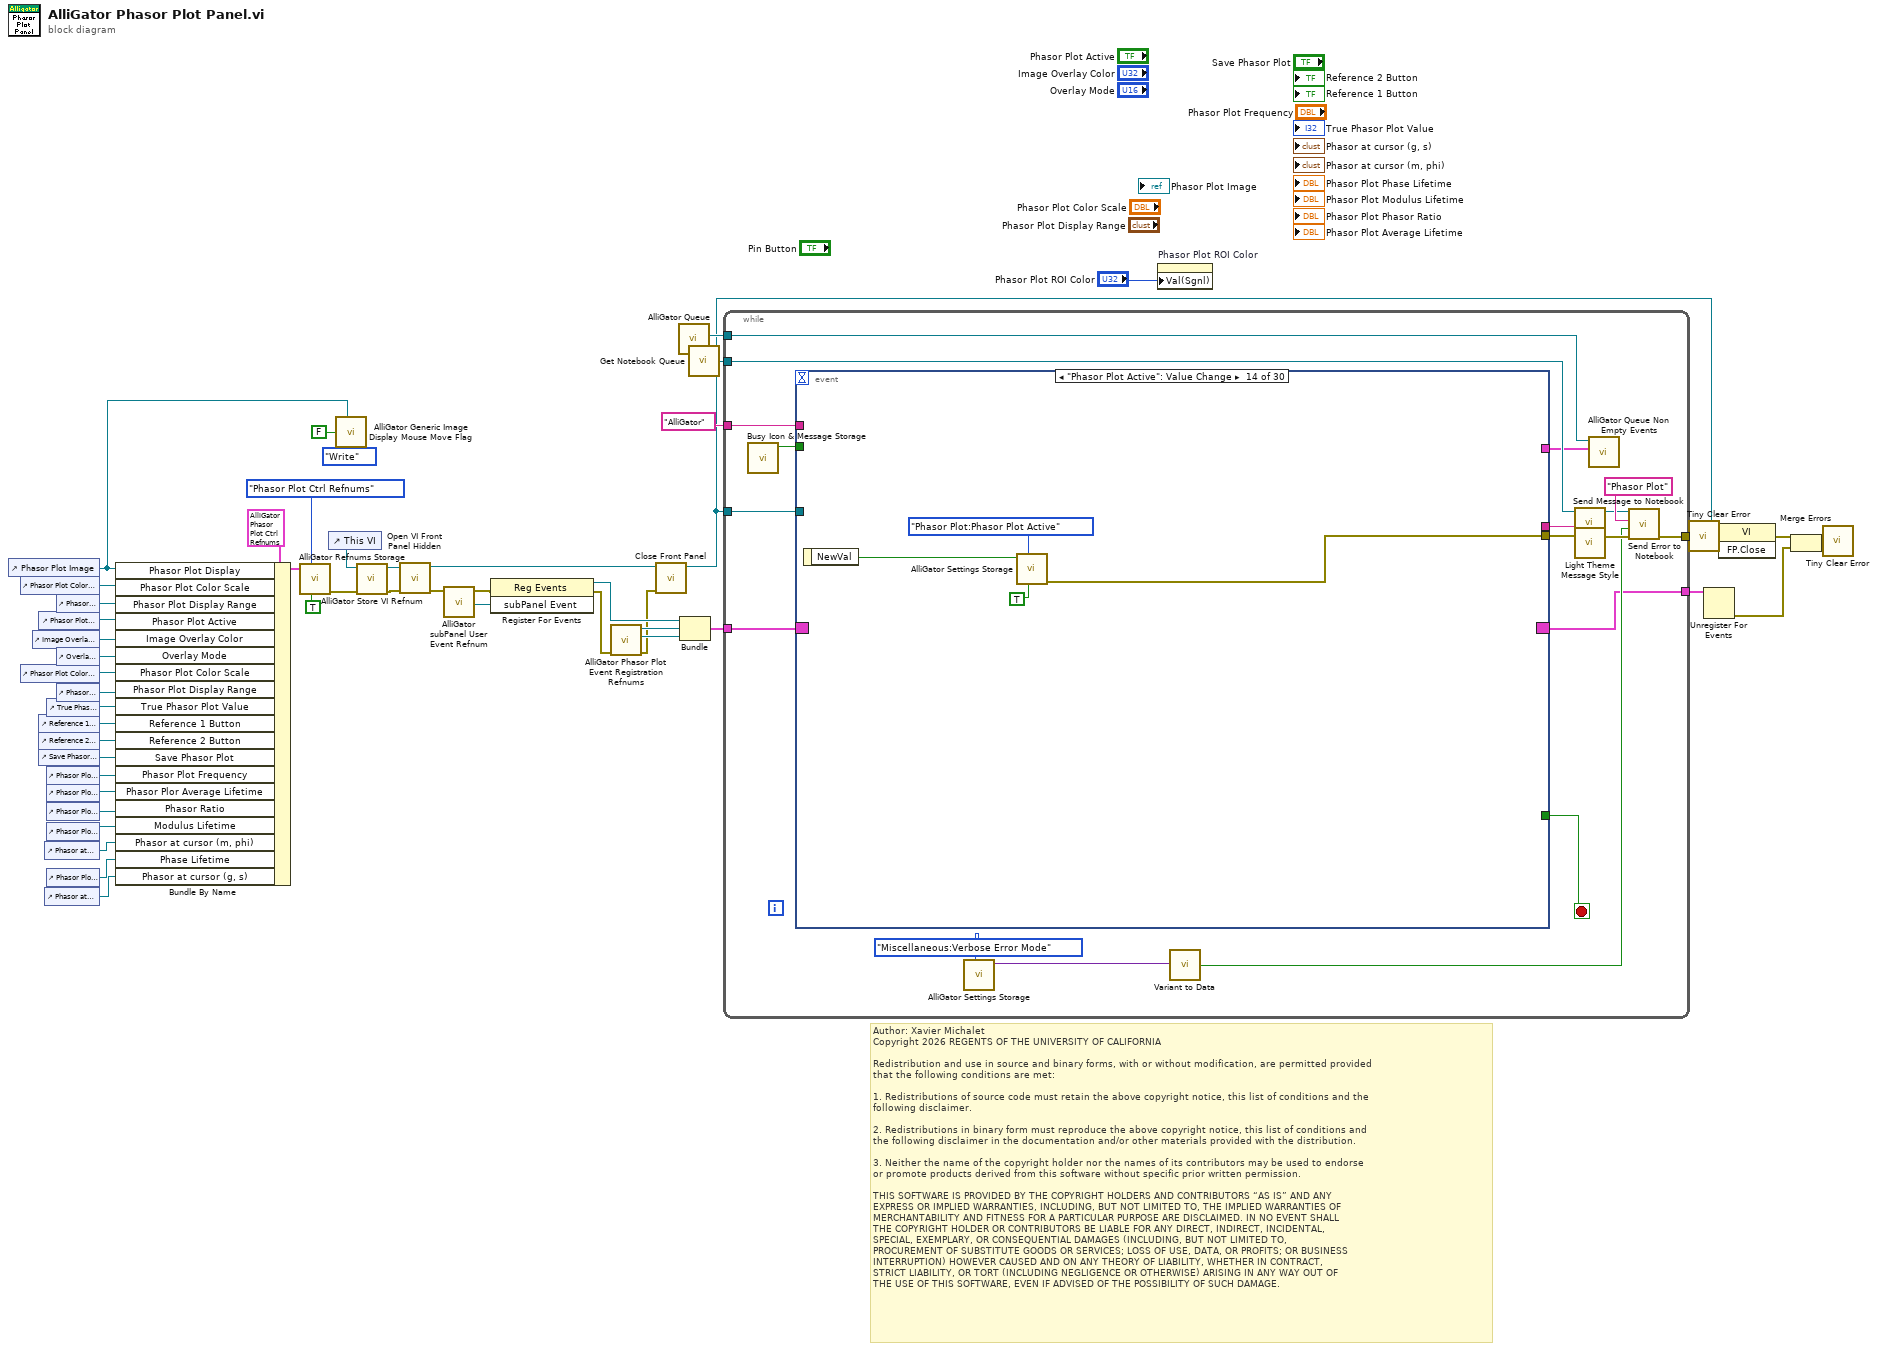
[diagram p0: block diagram]
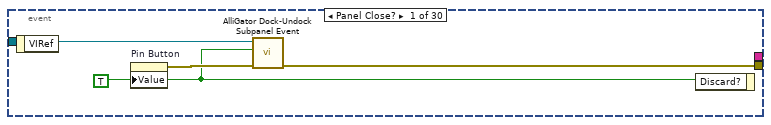
[diagram p2: hidden frame]
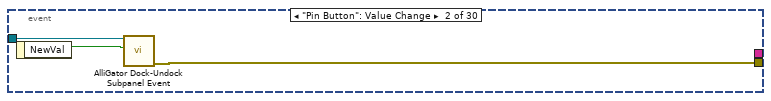
[diagram p3: hidden frame]
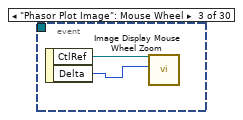
[diagram p4: hidden frame]
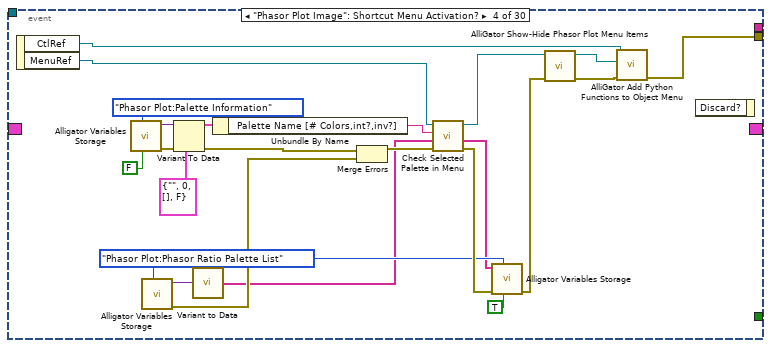
[diagram p5: hidden frame]
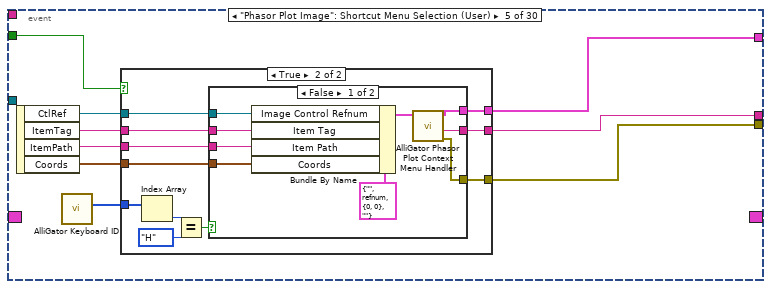
[diagram p6: hidden frame]
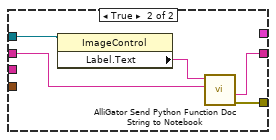
[diagram p8: hidden frame]
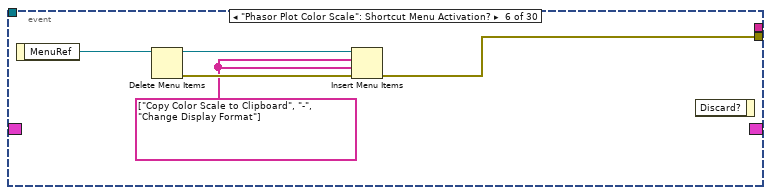
[diagram p9: hidden frame]
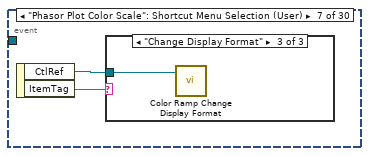
[diagram p10: hidden frame]
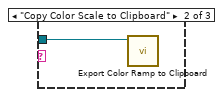
[diagram p12: hidden frame]
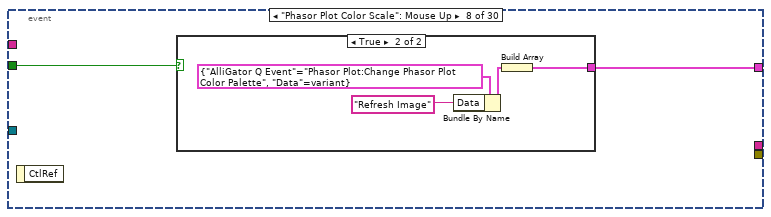
[diagram p13: hidden frame]
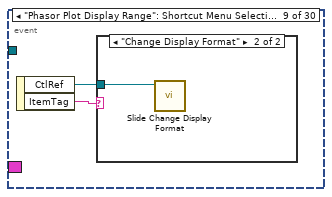
[diagram p15: hidden frame]
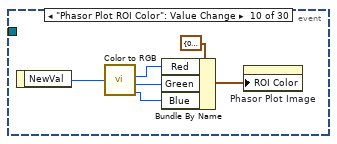
[diagram p17: hidden frame]
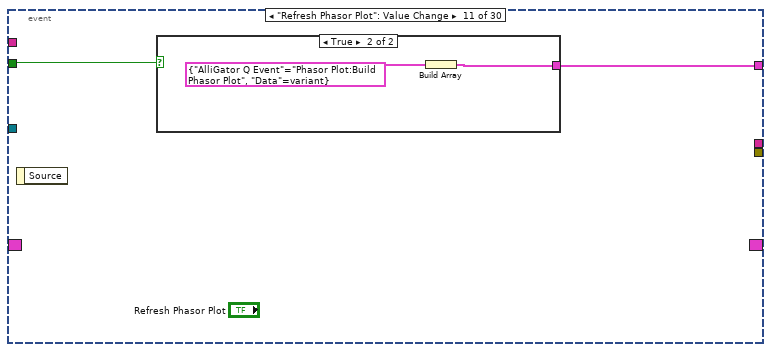
[diagram p18: hidden frame]
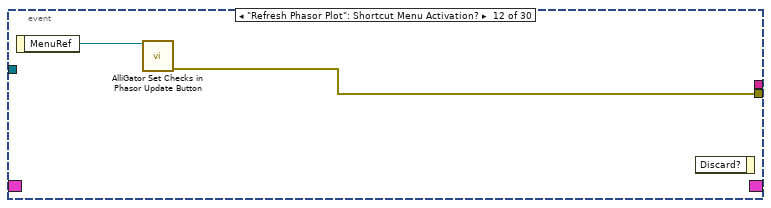
[diagram p20: hidden frame]
diagram:
  # "Author: Xavier Michalet\nCopyright 2026 REGENTS OF THE UNIVERSITY OF CALIFORNIA\n\nRedistribution and use in source and binary forms, with or without modification, are permitted provided\nthat the following conditions are met:\n\n1. Redistributions of source code must retain the above copyright notice, this list of conditions and the\nfollowing disclaimer.\n\n2. Redistributions in binary form must reproduce the above copyright notice, this list of conditions and\nthe following disclaimer in the documentation and/or other materials provided with the distribution.\n\n3. Neither the name of the copyright holder nor the names of its contributors may be used to endorse \nor promote products derived from this software without specific prior written permission.\n\nTHIS SOFTWARE IS PROVIDED BY THE COPYRIGHT HOLDERS AND CONTRIBUTORS “AS IS” AND ANY \nEXPRESS OR IMPLIED WARRANTIES, INCLUDING, BUT NOT LIMITED TO, THE IMPLIED WARRANTIES OF\nMERCHANTABILITY AND FITNESS FOR A PARTICULAR PURPOSE ARE DISCLAIMED. IN NO EVENT SHALL\nTHE COPYRIGHT HOLDER OR CONTRIBUTORS BE LIABLE FOR ANY DIRECT, INDIRECT, INCIDENTAL, \nSPECIAL, EXEMPLARY, OR CONSEQUENTIAL DAMAGES (INCLUDING, BUT NOT LIMITED TO, \nPROCUREMENT OF SUBSTITUTE GOODS OR SERVICES; LOSS OF USE, DATA, OR PROFITS; OR BUSINESS\nINTERRUPTION) HOWEVER CAUSED AND ON ANY THEORY OF LIABILITY, WHETHER IN CONTRACT, \nSTRICT LIABILITY, OR TORT (INCLUDING NEGLIGENCE OR OTHERWISE) ARISING IN ANY WAY OUT OF\nTHE USE OF THIS SOFTWARE, EVEN IF ADVISED OF THE POSSIBILITY OF SUCH DAMAGE."
  n1 = control-ref of="Phasor Plot Image"() -> (w6:refnum<vi>)
  n2 = control-ref of="Phasor Plot Color Scale"() -> (w34:refnum<vi>)
  n3 = control-ref of="Phasor Plot Color Scale"() -> (w26:refnum<vi>)
  n4 = control-ref of="Image Overlay Color"() -> (w28:refnum<vi>)
  n5 = control-ref of="Phasor Plot Active"() -> (w29:refnum<vi>)
  n6 = control-ref of="Reference 1 Button"() -> (w23:refnum<vi>)
  n7 = control-ref of="Reference 2 Button"() -> (w22:refnum<vi>)
  n8 = control-ref of="Save Phasor Plot"() -> (w21:refnum<vi>)
  n9 = control-ref of="Phasor at cursor (m, phi)"() -> (w16:refnum<vi>)
  n10 = control-ref of="Phasor at cursor (g, s)"() -> (w14:refnum<vi>)
  n11 = control-ref of="True Phasor Plot Value"() -> (w24:refnum<vi>)
  n12 = control-ref of="Phasor Plot Frequency"() -> (w20:refnum<vi>)
  n13 = control-ref of="Phasor Plot Average Lifetime"() -> (w19:refnum<vi>)
  n14 = control-ref of="Phasor Plot Phasor Ratio"() -> (w18:refnum<vi>)
  n15 = control-ref of="Phasor Plot Modulus Lifetime"() -> (w17:refnum<vi>)
  n16 = control-ref of="Phasor Plot Phase Lifetime"() -> (w15:refnum<vi>)
  n17 = control-ref of="Phasor Plot Display Range"() -> (w33:refnum<vi>)
  n18 = control-ref of="Overlay Mode"() -> (w27:refnum<vi>)
  n19 = control-ref of="Phasor Plot Display Range"() -> (w25:refnum<vi>)
  n20 = Bundle By Name(cluster=T6 {"Phasor Ratio"=refnum, "Modulus Lifetime"=refnum, "Phasor at cursor (m, phi)"=refnum, "Phase Lifetime"=refnum, "Phasor at cursor (g, s)"=refnum, "Phasor Plor Average Lifetime"=refnum, "Phasor Plot Active"=refnum, "Save Phasor Plot"=refnum, "Image Overlay Color"=refnum, "Phasor Plot Color Scale"=refnum, "Reference 1 Button"=refnum, "Reference 2 Button"=refnum, "True Phasor Plot Value"=refnum, "Phasor Plot Display Range"=refnum, "Phasor Plot Display"=refnum, "Phasor Plot Frequency"=refnum, "Overlay Mode"=refnum} ("Phasor Plot Ctrl Refnums"), "Phasor Plot Display"=w6, "Phasor Plot Color Scale"=w34, "Phasor Plot Display Range"=w33, "Phasor Plot Active"=w29, "Image Overlay Color"=w28, "Overlay Mode"=w27, "Phasor Plot Color Scale"=w26, "Phasor Plot Display Range"=w25, "True Phasor Plot Value"=w24, "Reference 1 Button"=w23, "Reference 2 Button"=w22, "Save Phasor Plot"=w21, "Phasor Plot Frequency"=w20, "Phasor Plor Average Lifetime"=w19, "Phasor Ratio"=w18, "Modulus Lifetime"=w17, "Phasor at cursor (m, phi)"=w16, "Phase Lifetime"=w15, "Phasor at cursor (g, s)"=w14) -> (w39:T6)
  n21 = call "AlliGator Refnums Storage.vi"("Get(F)/Set"=TRUE, "AlliGator Refnum List"=AlliGator_Refnums_List."Phasor Plot Ctrl Refnums", "Data in"=w39) -> ("Error Out"=w2:errorcluster)  [unwired: 7 in, 1 out]
  n22 = control-ref of="This VI"() -> (w3:refnum<vi>)
  n23 = call "AlliGator Generic Image Display Mouse Move Flag.vi"("Image Control Refnum"=w6, "Flag (in)"=FALSE, "Read/Write"=Read-Write."Write") -> ()  [unwired: 6 in, 1 out]
  n24 = call "AlliGator Store VI Refnum.vi"("error in (no error)"=w2, "VI Refnum"=w3) -> ("error out"=w5:errorcluster, "VI Refnum (dup)"=w1:refnum<vi>)  [unwired: 7 in, 1 out]
  n25 = call "Open VI Front Panel Hidden.vi"("error in"=w5, "VI in"=w1) -> ("error out"=w13:errorcluster, "VI out"=w11:refnum<vi>)  [unwired: 8 in]
  n26 = call "AlliGator subPanel User Event Refnum.vi"() -> ("subPanel Event"=w46:refnum<user-event>)  [unwired: 9 in]
  n27 = register-events(error in=w13, w46) -> (reference out=w45:refnum<event-registration>, error out=w12:errorcluster)  [unwired: 1 in]
  n28 = call "AlliGator Phasor Plot Event Registration Refnums.vi"("error in (no error)"=w12) -> ("error out"=w10:errorcluster, "Phasor Plote Display Range Event"=w30:refnum<event-registration>, "Phasor Plot Display Event"=w31:refnum<event-registration>)  [unwired: 8 in]
  n29 = call "Close Front Panel.vi"("error in (no error)"=w10, "VI in"=w11) -> ("VI out"=w9:refnum<vi>)  [unwired: 8 in, 1 out]
  n30 = call "AlliGator Queue.vi"() -> ("AlliGator Q"=w48:refnum<queue>)  [unwired: 8 in, 1 out]
  n31 = Bundle("Event Registration Refnum"=w45, "Phasor Plot Display Event"=w31, "Phasor Plote Display Range Event"=w30) -> (w38:T7)  [unwired: 1 in]
  n32 = call "Get Notebook Queue.vi"() -> ("Notebook Queue"=w49:refnum<queue>)  [unwired: 9 in]
  n33 = while {
    tunnel: w49 -> [w60]
    tunnel: w48 -> [w57]
    tunnel: "AlliGator" ("Sender") -> [w55]
    tunnel: w9 -> [w53]
    tunnel: w38 -> [w52]
    tunnel: [w51] -> w44
    tunnel: [w50] -> w43
    stop <- w67 stop-if-true
    n34 = call "Busy Icon & Message Storage.vi"() -> ("Busy Icon Status (F = busy)"=w54:bool)  [unwired: 9 in, 2 out]
    n35 = event shown="[13] \"Phasor Plot Active\": Value Change" {
      selector: w52 -> [_ _ _ _ _ _ _ _ _ _ _ _ _ _ _ _ _ _ _ _ _ _ w230 w257 w270 _ w307 w343 w349 _]
      dyn-events: [_ _ _ _ _ _ _ _ _ _ _ _ _ _ _ _ _ _ _ _ _ _ w229 w255 w269 _ w306 w343 w348 _] -> w51
      timeout: _ -> [_ _ _ _ _ _ _ _ _ _ _ _ _ _ _ _ _ _ _ _ _ _ _ _ _ _ _ _ _ _]
      tunnel: [w69 w72 _ w77 w100 w134 _ _ _ _ _ w162 w164 w168 w172 w205 _ _ w214 w216 _ _ w228 w254 w268 _ w305 w342 w347 _] -> w61
      tunnel: [_ _ _ _ _ _ _ _ _ _ _ _ _ _ _ _ _ _ _ _ _ w221 _ _ _ _ _ _ _ _] -> w67
      tunnel: [_ _ _ _ w101 _ _ _ _ _ _ _ _ _ w171 _ _ _ _ _ _ _ _ _ _ _ _ _ _ _] -> w58
      tunnel: [_ _ _ _ w102 _ _ w144 _ _ w159 _ _ _ w175 _ w209 w212 _ _ w219 _ _ _ _ w280 w304 _ _ w353] -> w56
      tunnel: w54 -> [_ _ _ _ w104 _ _ w143 _ _ w158 _ _ _ _ _ w208 w211 _ _ w218 _ w227 w253 w266 w281 w308 _ _ w354]
      tunnel: w55 -> [_ _ _ _ _ _ _ _ _ _ _ _ _ _ w174 _ _ _ _ _ _ _ _ _ _ _ _ _ _ _]
      tunnel: w53 -> [_ w74 _ _ _ _ _ _ _ _ _ _ _ _ _ _ _ _ _ _ _ _ _ _ _ _ _ _ _ _]
      event Panel Close? {
        w68 = TRUE ("Pin Button")
        n36 = event-data() -> ("VIRef"=w71:refnum<vi>)  [unwired: 1 in]
        n37 = property on="Pin Button" class="Bool (strict)"("Value"=w68) -> (error out=w70:errorcluster)  [unwired: 2 in, 1 out]
        n38 = call "AlliGator Dock-Undock Subpanel Event.vi"("Error In"=w70, "Dock?"=w68, "VI in"=w71) -> ("Error Out"=w69:errorcluster)  [unwired: 8 in]
        n39 = event-data("Discard?"=w68) -> ()  [unwired: 1 in, 1 out]
      }
      event "Pin Button": Value Change {
        n40 = event-data() -> ("NewVal"=w73:bool)  [unwired: 1 in]
        n41 = call "AlliGator Dock-Undock Subpanel Event.vi"("Dock?"=w73, "VI in"=w74) -> ("Error Out"=w72:errorcluster)  [unwired: 9 in]
      }
      event "Phasor Plot Image": Mouse Wheel {
        n42 = event-data() -> ("CtlRef"=w76:refnum<vi>, "Delta"=w75:i32)  [unwired: 1 in]
        n43 = call "Image Display Mouse Wheel Zoom.vi"("Mouse Wheel Delta"=w75, "Image Control Refnum"=w76) -> ()  [unwired: 9 in, 1 out]
      }
      event "Phasor Plot Image": Shortcut Menu Activation? {
        w92 = AlliGator_Variables_List."Phasor Plot:Phasor Ratio Palette List" ("Alligator Variable")
        n44 = event-data() -> ("CtlRef"=w79:refnum<vi>, "MenuRef"=w78:refnum<k9>)  [unwired: 1 in]
        n45 = call "Alligator Variables Storage.vi"("Get(F)/Set"=FALSE, "AlliGator Variable"=AlliGator_Variables_List."Phasor Plot:Palette Information" ("Alligator Variable")) -> ("Error Out"=w83:errorcluster, "Data out"=w82:variant)  [unwired: 7 in, 1 out]
        n46 = call "Alligator Variables Storage.vi"("AlliGator Variable"=w92) -> ("Error Out"=w97:errorcluster, "Data out"=w88:variant)  [unwired: 8 in, 1 out]
        n47 = Variant To Data(error in=w83, type=T9 {"Palette Name [# Colors,int?,inv?]"="", "Palette Type"=0, "Palette Colors"=[], "Interpolate?"=FALSE} ("Image Display Palette Information"), Variant=w82) -> (data=w84:T9, error out=w85:errorcluster)
        n48 = call-poly "Variant to Data.vi"("Variant"=w88) -> ("String Array"=w89:string[])  [unwired: 8 in]
        n49 = Unbundle By Name(w84) -> ("Palette Name [# Colors,int?,inv?]"=w87:string)
        n50 = Merge Errors(w85, w97) -> (w96:errorcluster)
        n51 = call "Check Selected Palette in Menu.vi"("Error In"=w96, "Palette List"=w89, "Checked Palette"=w87, "Menu in"=w78) -> ("Error Out"=w93:errorcluster, "Stored Palette List"=w91:string[], "menu reference out"=w94:refnum<k9>)  [unwired: 5 in]
        n52 = call "Alligator Variables Storage.vi"("Get(F)/Set"=TRUE, "AlliGator Variable"=w92, "Error In"=w93, "Data in"=w91) -> ("Error Out"=w95:errorcluster)  [unwired: 5 in, 2 out]
        n53 = call "AlliGator Show-Hide Phasor Plot Menu Items.vi"("error in (no error)"=w95, "Menu in"=w94) -> ("error out"=w98:errorcluster, "Menu out"=w99:refnum<k9>)  [unwired: 8 in]
        n54 = call "AlliGator Add Python Functions to Object Menu.vi"("error in (no error)"=w98, "Menu in"=w99, "Object Refnum"=w79) -> ("error out"=w77:errorcluster)  [unwired: 6 in, 2 out]
        n55 = event-data() -> ()  [unwired: 2 in, 1 out]
      }
      event "Phasor Plot Image": Shortcut Menu Selection (User) {
        n56 = event-data() -> ("CtlRef"=w108:refnum<vi>, "ItemTag"=w107:string, "ItemPath"=w106:string, "Coords"=w105:T15)  [unwired: 1 in]
        n57 = call "AlliGator Keyboard ID.vi"() -> ("keys pressed"=w103:T24)  [unwired: 9 in, 2 out]
        n58 = case shown="True" w104 {
          tunnel: w105 -> [_ w119]
          tunnel: w106 -> [_ w118]
          tunnel: w108 -> [_ w117]
          tunnel: w107 -> [_ w116]
          tunnel: [_ w115] -> w102
          tunnel: w103 -> [_ w111]
          tunnel: [_ w110] -> w101
          tunnel: [_ w109] -> w100
          frame False {
          }
          frame True {
            n59 = Index Array(array=w111) -> (element=w114:T12)  [unwired: 1 in]
            n60 = Equal?(x=w114, y=T12."H" ("element")) -> (x = y?=w112:bool)
            n61 = case shown="False" w112 {
              tunnel: w119 -> [w128 _]
              tunnel: w118 -> [w127 _]
              tunnel: w117 -> [w126 w132]
              tunnel: w116 -> [w125 w131]
              tunnel: [w124 _] -> w115
              tunnel: [w121 w130] -> w110
              tunnel: [w120 w129] -> w109
              frame False {
                n62 = Bundle By Name(cluster=T13 {"Item Tag"="", "Image Control Refnum"=refnum, "Coords"={"Horizontal"=0, "Vertical"=0}, "Item Path"=""} ("Image Event Data"), "Image Control Refnum"=w126, "Item Tag"=w125, "Item Path"=w127, "Coords"=w128) -> (w122:T13)
                n63 = call "AlliGator Phasor Plot Context Menu Handler.vi"("Image Event"=w122) -> ("Error Out"=w120:errorcluster, "Message"=w121:string, "AlliGator Actions"=w124:T16[])  [unwired: 8 in]
              }
              frame True {
                n64 = property class="ImageControl"(reference=w132) -> ("Label.Text"=w133:string)  [unwired: 1 in, 2 out]
                n65 = call "AlliGator Send Python Function Doc String to Notebook.vi"("Item Tag"=w131, "Target"=w133) -> ("Error Out"=w129:errorcluster, "Message"=w130:string)  [unwired: 8 in]
              }
            }
          }
        }
      }
      event "Phasor Plot Color Scale": Shortcut Menu Activation? {
        w137 = string[] ["Copy Color Scale to Clipboard", "-", "Change Display Format"] ("item names")
        n66 = event-data() -> ("MenuRef"=w135:refnum<k9>)  [unwired: 1 in]
        n67 = Delete Menu Items(9:w135) -> (0:w138:errorcluster, 3:w136:refnum<k9>)  [unwired: 3 in]
        n68 = Insert Menu Items(6:w138, 7:w137, 8:w137, 9:w136) -> (0:w134:errorcluster)  [unwired: 2 in, 2 out]
        n69 = event-data() -> ()  [unwired: 2 in, 1 out]
      }
      event "Phasor Plot Color Scale": Shortcut Menu Selection (User) {
        n70 = event-data() -> ("CtlRef"=w140:refnum<vi>, "ItemTag"=w139:string)  [unwired: 1 in]
        n71 = case shown="\"Change Display Format\"" w139 {
          tunnel: w140 -> [_ w141 w142]
          frame "", Default {
          }
          frame "Copy Color Scale to Clipboard" {
            n72 = call "Export Color Ramp to Clipboard.vi"("ColorRamp Refnum"=w141) -> ()  [unwired: 11 in]
          }
          frame "Change Display Format" {
            n73 = call "Color Ramp Change Display Format.vi"("ColorRamp Refnum"=w142) -> ()  [unwired: 10 in, 1 out]
          }
        }
      }
      event "Phasor Plot Color Scale": Mouse Up {
        n74 = event-data() -> ()  [unwired: 1 in, 1 out]
        n75 = case shown="True" w143 {
          tunnel: [_ w145] -> w144
          frame False {
          }
          frame True {
            n76 = Bundle By Name(cluster=T16 {"AlliGator Q Event"=enum."Phasor Plot:Change Phasor Plot Color Palette", "Data"=variant} ("element"), "Data"="Refresh Image" ("String")) -> (w147:T16)
            n77 = Build Array(w147) -> (w145:T16[])
          }
        }
      }
      event "Phasor Plot Display Range": Shortcut Menu Selection (User) {
        n78 = event-data() -> ("CtlRef"=w150:refnum<vi>, "ItemTag"=w149:string)  [unwired: 1 in]
        n79 = case shown="\"Change Display Format\"" w149 {
          tunnel: w150 -> [_ w151]
          frame "", Default {
          }
          frame "Change Display Format" {
            n80 = call "Slide Change Display Format.vi"("Slide Refnum"=w151) -> ()  [unwired: 10 in, 1 out]
          }
        }
      }
      event "Phasor Plot ROI Color": Value Change {
        n81 = event-data() -> ("NewVal"=w153:u32)  [unwired: 1 in]
        n82 = call <vilib>:"Color to RGB.vi"("Color"=w153) -> ("R"=w156:u8, "G"=w155:u8, "B"=w154:u8)  [unwired: 1 out]
        n83 = Bundle By Name(cluster=cluster{"Red":u8, "Green":u8, "Blue":u8} {"Red"=0, "Green"=0, "Blue"=0} ("ROI Color"), "Red"=w156, "Green"=w155, "Blue"=w154) -> (w152:cluster{"Red":u8, "Green":u8, "Blue":u8})
        n84 = property on="Phasor Plot Image" class="ImageControl"("ROI Color"=w152) -> ()  [unwired: 2 in, 2 out]
      }
      event "Refresh Phasor Plot": Value Change {
        n85 = event-data() -> ()  [unwired: 1 in, 1 out]
        n86 = case shown="True" w158 {
          tunnel: [_ w160] -> w159
          frame False {
          }
          frame True {
            n87 = Build Array(T16 {"AlliGator Q Event"=enum."Phasor Plot:Build Phasor Plot", "Data"=variant} ("Time-Gated Phasor Q Element")) -> (w160:T16[])
          }
        }
      }
      event "Refresh Phasor Plot": Shortcut Menu Activation? {
        n88 = event-data() -> ("MenuRef"=w163:refnum<k9>)  [unwired: 1 in]
        n89 = call "AlliGator Set Checks in Phasor Update Button.vi"("Menu in"=w163) -> ("Error Out"=w162:errorcluster)  [unwired: 10 in]
        n90 = event-data() -> ()  [unwired: 2 in, 1 out]
      }
      event "Refresh Phasor Plot": Shortcut Menu Selection (User) {
        n91 = event-data() -> ("ItemTag"=w166:string, "CtlRef"=w165:refnum<vi>)  [unwired: 1 in]
        n92 = call "AlliGator Update Phasor Image Elements to Update.vi"("CtlRef"=w165, "Phasor Plot Element to Update"=w166) -> ("Error Out"=w164:errorcluster)  [unwired: 8 in, 1 out]
      }
      event "Phasor Plot Active": Value Change {
        n93 = event-data() -> ("NewVal"=w167:bool)  [unwired: 1 in]
        n94 = call "AlliGator Settings Storage.vi"("Get(F)/Set"=TRUE, "AlliGator Settings List"=AlliGator_Settings_List."Phasor Plot:Phasor Plot Active", "Variant Data in"=w167) -> ("Error Out"=w168:errorcluster)  [unwired: 7 in, 1 out]
      }
      event "Save Phasor Plot", "Phasor Plot Frequency": Value Change {
        n95 = event-data() -> ("CtlRef"=w176:refnum<vi>, "NewVal"=w173:variant)  [unwired: 1 in]
        n96 = property class="Ctl"(reference=w176) -> (reference out=w180:refnum<vi>, error out=w177:errorcluster, "Label.Text"=w181:string)  [unwired: 1 in]
        n97 = case shown="\"Phasor Plot Frequency\"" w181 {
          tunnel: w177 -> [w182 w189]
          tunnel: [w182 w193] -> w178
          tunnel: [_ T16[] [{"AlliGator Q Event"=enum."Phasor Graph:Update SEPL Plot", "Data"=variant}] ("element")] -> w175
          tunnel: w174 -> [_ w195]
          tunnel: w173 -> [_ w191]
          frame "", Default {
            # "only updates the corresponding Settings window control"
          }
          frame "Phasor Plot Frequency" {
            # "Need to update TWO controls"
            n98 = call "AlliGator Phasor Graph Ctrl Refnums.vi"() -> ("error out"=w184:errorcluster, "Phasor Graph Ctrl Refnums"=w187:T25)  [unwired: 10 in]
            n99 = Variant To Data(error in=w189, type=dbl[unit] 0.0 ("Calibration Phasor Frequency"), Variant=w191) -> (data=w185:dbl[unit], error out=w188:errorcluster)
            n100 = Unbundle By Name(w187) -> ("Phasor Graph Frequency"=w186:refnum<vi>)
            n101 = call "Alligator Variables Storage.vi"("AlliGator Variable"=AlliGator_Variables_List."Phasor Plot:Computed" ("Alligator Variable"), "Error In"=w189) -> ("Error Out"=w194:errorcluster, "Data out"=w198:variant)  [unwired: 7 in, 1 out]
            n102 = call "AlliGator Update Settings & Control.vi"("Error In"=w188, "Value"=w185, "Sender"=w195, "CtlRef"=w186) -> ("Error Out"=w192:errorcluster)  [unwired: 7 in]
            n103 = call-poly "Variant to Data.vi"("Variant"=w198) -> ("Value"=w197:bool)  [unwired: 8 in]
            n104 = case shown="True" w197 {
              tunnel: w194 -> [w201 w204]
              tunnel: [w201 w202] -> w200
              frame False {
              }
              frame True {
                n105 = call "AlliGator Set Phasor Plot Update LED.vi"("error in (no error)"=w204, "Off/On"=TRUE) -> ("error out"=w202:errorcluster)  [unwired: 9 in]
              }
            }
            n106 = property class="DigNum (strict)"(reference=w186, error in=w184, "Value"=w185) -> (error out=w183:errorcluster)  [unwired: 1 out]
            n107 = Merge Errors(w200, w192, w183) -> (w193:errorcluster)
          }
        }
        n108 = call "AlliGator Update Settings & Control.vi"("Error In"=w178, "Value"=w173, "Sender"=w174, "CtlRef"=w180) -> ("Error Out"=w179:errorcluster)  [unwired: 7 in]
        n109 = call "AlliGator Get Control Notebook String.vi"("error in (no error)"=w179, "Value"=w173, "Control Label"=w181) -> ("error out"=w172:errorcluster, "Notebook String"=w171:string)  [unwired: 7 in]
      }
      event "Phasor Plot Frequency": Shortcut Menu Selection (User) {
        n110 = event-data() -> ("CtlRef"=w207:refnum<vi>, "ItemTag"=w206:string)  [unwired: 1 in]
        n111 = call "AlliGator Set Special Phasor Frequency.vi"("ItemTag"=w206, "Frequency Refnum"=w207) -> ("error out"=w205:errorcluster)  [unwired: 9 in]
      }
      event "Phasor ROI Decay": Value Change {
        n112 = event-data() -> ()  [unwired: 1 in, 1 out]
        n113 = case shown="True" w208 {
          tunnel: [_ T16[] [{"AlliGator Q Event"=enum."Phasor Plot:Compute Decay of Selected Phasors", "Data"=variant}] ("element")] -> w209
          frame False {
          }
          frame True {
          }
        }
      }
      event "Clear Phasor Overlay": Value Change {
        n114 = event-data() -> ()  [unwired: 1 in, 1 out]
        n115 = case shown="True" w211 {
          tunnel: [_ T16[] [{"AlliGator Q Event"=enum."Phasor Plot:Clear Phasor Overlay", "Data"=variant}] ("element")] -> w212
          frame False {
          }
          frame True {
          }
        }
      }
      event "Clear Phasor Overlay": Shortcut Menu Activation? {
        n116 = event-data() -> ("MenuRef"=w215:refnum<k9>)  [unwired: 1 in]
        n117 = call "AlliGator Set Checkmarks in Phasor Overlay to Erase Button Menu.vi"("Menu in"=w215) -> ("Error Out"=w214:errorcluster)  [unwired: 10 in]
        n118 = event-data() -> ()  [unwired: 2 in, 1 out]
      }
      event "Clear Phasor Overlay": Shortcut Menu Selection (User) {
        n119 = event-data() -> ("ItemTag"=w217:string)  [unwired: 1 in]
        n120 = call "AlliGator Update Checkmarks in Phasor Overlay to Erase Button Menu.vi"("Phasor Plot Overlay to Erase"=w217) -> ("Error Out"=w216:errorcluster)  [unwired: 10 in]
      }
      event "Highlight Phasor in Source Image": Value Change {
        n121 = event-data() -> ()  [unwired: 1 in, 1 out]
        n122 = case shown="True" w218 {
          tunnel: [_ T16[] [{"AlliGator Q Event"=enum."Phasor Plot:Overlay Phasor ROI, Ratio or Map in Source Image", "Data"=variant}] ("element")] -> w219
          frame False {
          }
          frame True {
          }
        }
      }
      event User Event {
        n123 = event-data() -> ("subpanel"=w223:string, "event"=w222:string)  [unwired: 1 in]
        n124 = case shown="\"AlliGator\"" w223 {
          tunnel: w222 -> [_ w225]
          tunnel: [_ w224] -> w221
          frame "False", Default {
          }
          frame "AlliGator" {
            n125 = case shown="\"False\", Default" w225 {
              tunnel: [_ TRUE] -> w224
              frame "False", Default {
              }
              frame "quit" {
              }
            }
          }
        }
      }
      event Mouse Down {
        n126 = event-data() -> ("CtlRef"=w235:refnum<vi>, "Coords"=w234:T15, "Button"=w233:u16, "PlatMods.Shift"=w232:bool, "PlatMods.Alt"=w231:bool)  [unwired: 1 in]
        n127 = case shown="True" w227 {
          tunnel: w235 -> [_ w244]
          tunnel: w234 -> [_ w243]
          tunnel: w233 -> [_ w242]
          tunnel: w230 -> [w236 w241]
          tunnel: [w236 w240] -> w229
          tunnel: w232 -> [_ w239]
          tunnel: w231 -> [_ w238]
          tunnel: [_ w237] -> w228
          frame False {
          }
          frame True {
            n128 = case shown="1" w242 {
              tunnel: w244 -> [_ w250]
              tunnel: w243 -> [_ _]
              tunnel: w241 -> [w245 w251]
              tunnel: [w245 w252] -> w240
              tunnel: w239 -> [_ _]
              tunnel: w238 -> [_ _]
              tunnel: [_ w249] -> w237
              frame 0, Default {
                # "right or middle button"
              }
              frame 1 {
                # "Left Button: look for mouse up"
                n129 = Unbundle By Name(w251) -> ("Phasor Plot Display Event"=w248:refnum<event-registration>)
                n130 = call "AlliGator Phasor Plot Display Mouse Down-Up Event Monitoring.vi"("Phasor Plot Display Event Registration"=w248, "Phasor Plot Display Refnum"=w250, "Look for Mouse Down(T)/Up(F)"=FALSE) -> ("Phasor Plot Display Event Registration"=w247:refnum<event-registration>, "Error Out"=w249:errorcluster)  [unwired: 11 in]
                n131 = Bundle By Name(cluster=w251, "Phasor Plot Display Event"=w247) -> (w252:T7)
              }
            }
          }
        }
      }
      event Mouse Enter {
        n132 = event-data() -> ("CtlRef"=w256:refnum<vi>)  [unwired: 1 in]
        n133 = case shown="True" w253 {
          tunnel: [w258 w263] -> w255
          tunnel: w257 -> [w258 w262]
          tunnel: w256 -> [_ w259]
          tunnel: [_ w260] -> w254
          frame False {
          }
          frame True {
            n134 = Unbundle By Name(w262) -> ("Phasor Plot Display Event"=w264:refnum<event-registration>)
            n135 = register-events(reference=w264, T14 refnum ("event source"), w259, w259, w259, w259) -> (reference out=w265:refnum<event-registration>, error out=w260:errorcluster)  [unwired: 1 in]
            n136 = Bundle By Name(cluster=w262, "Phasor Plot Display Event"=w265) -> (w263:T7)
          }
        }
      }
      event Mouse Leave {
        n137 = event-data() -> ("CtlRef"=w267:refnum<vi>)  [unwired: 1 in]
        n138 = case shown="True" w266 {
          tunnel: [w271 w277] -> w269
          tunnel: w270 -> [w271 w276]
          tunnel: w267 -> [_ w275]
          tunnel: [_ w272] -> w268
          frame False {
          }
          frame True {
            w274 = refnum<vi> refnum ("event source")
            n139 = Unbundle By Name(w276) -> ("Phasor Plot Display Event"=w278:refnum<event-registration>)
            n140 = register-events(reference=w278, w275, w274, w274, w274, w274) -> (reference out=w279:refnum<event-registration>, error out=w273:errorcluster)  [unwired: 1 in]
            n141 = Bundle By Name(cluster=w276, "Phasor Plot Display Event"=w279) -> (w277:T7)
            n142 = call "AlliGator Show-Hide Phasor Indicators.vi"("Error In"=w273) -> ("Error Out"=w272:errorcluster)  [unwired: 10 in]
          }
        }
      }
      event Mouse Move {
        n143 = event-data() -> ("Time"=w283:u32, "CtlRef"=w282:refnum<vi>)  [unwired: 1 in]
        n144 = case shown="True" w281 {
          tunnel: w282 -> [_ w284]
          tunnel: [_ w291] -> w280
          tunnel: w283 -> [_ w286]
          frame False {
          }
          frame True {
            w285 = T16 {"AlliGator Q Event"=enum."Phasor Plot:Mouse Move", "Data"=variant} ("AlliGator Actions")
            n145 = call "AlliGator Filter Event.vi"("Time"=w286, "AlliGatorr Q Element"=w285) -> ("Filter Event?"=w287:bool)  [unwired: 8 in, 1 out]
            n146 = call "AlliGator Generic Image Display Mouse Move Flag.vi"("Image Control Refnum"=w284, "Read/Write"=Read-Write."Read") -> ("Flag (out)"=w288:bool)  [unwired: 7 in]
            n147 = Compound Arithmetic op=OR(w287, w288) -> (w289:bool)
            n148 = case shown="False" w289 {
              tunnel: w284 -> [w302 _]
              tunnel: [w299 _] -> w291
              tunnel: w285 -> [w297 _]
              frame False {
                n149 = property class="ImageControl"(reference=w302) -> (reference out=w294:refnum<vi>, "Last Mouse Position"=w298:cluster{"X":i32, "Y":i32})  [unwired: 1 in, 1 out]
                n150 = call "AlliGator Mouse ID.vi"() -> ("button info"=w292:T26)  [unwired: 8 in, 3 out]
                n151 = call "AlliGator Keyboard ID.vi"() -> ("keys pressed"=w293:T24)  [unwired: 9 in, 2 out]
                n152 = call "AlliGator Generic Image Display Mouse Move Flag.vi"("Image Control Refnum"=w294, "Flag (in)"=TRUE, "Read/Write"=Read-Write."Write") -> ()  [unwired: 6 in, 1 out]
                n153 = Bundle(cluster=T18 {"Image Control Refnum"=refnum, "Coords"={"Horizontal"=0, "Vertical"=0}, "button info"={"button 1"=FALSE, "button 2"=FALSE, "button 3"=FALSE, "button 4"=FALSE}, "keys pressed"=[]} ("Image User Event Data"), "Image Control Refnum"=w294, "Coords"=w298, "button info"=w292, "keys pressed"=w293) -> (w300:T18)
                n154 = Bundle By Name(cluster=w297, "Data"=w300) -> (w303:T16)
                n155 = Build Array(w303) -> (w299:T16[])
              }
              frame True {
              }
            }
          }
        }
      }
      event Mouse Up {
        n156 = event-data() -> ("CtlRef"=w312:refnum<vi>, "Button"=w311:u16, "PlatMods.Shift"=w310:bool, "PlatMods.Alt"=w309:bool)  [unwired: 1 in]
        n157 = case shown="True" w308 {
          tunnel: w312 -> [_ w321]
          tunnel: w310 -> [_ w320]
          tunnel: w311 -> [_ w314]
          tunnel: w307 -> [w313 w319]
          tunnel: [w313 w318] -> w306
          tunnel: w309 -> [_ w317]
          tunnel: [_ w316] -> w305
          tunnel: [_ w315] -> w304
          frame False {
          }
          frame True {
            n158 = case shown="1" w314 {
              tunnel: w321 -> [_ w336]
              tunnel: w320 -> [_ w325]
              tunnel: w319 -> [w322 w334]
              tunnel: [w322 w339] -> w318
              tunnel: w317 -> [_ w324]
              tunnel: [_ w331] -> w316
              tunnel: [_ w327] -> w315
              frame 0, Default {
              }
              frame 1 {
                w335 = TRUE  # Look for Mouse Down
                # "Left Button"
                n159 = Unbundle By Name(w334) -> ("Phasor Plot Display Event"=w338:refnum<event-registration>)
                n160 = property class="ImageControl"(reference=w336) -> (reference out=w323:refnum<vi>, error out=w331:errorcluster, "Current ROI Tool"=w333:u32, "ROI"=w326:T27)  [unwired: 1 in]
                n161 = call "AlliGator Phasor Plot Display Mouse Down-Up Event Monitoring.vi"("Phasor Plot Display Event Registration"=w338, "Phasor Plot Display Refnum"=w336, "Look for Mouse Down(T)/Up(F)"=w335) -> ("Phasor Plot Display Event Registration"=w337:refnum<event-registration>)  [unwired: 11 in, 1 out]
                n162 = Bundle By Name(cluster=T19 {"Current ROI Tool"=8, "ROI Descriptor"={"Global Rectangle"=[], "Contours"=[]}, "Shift"=FALSE, "Alt"=FALSE, "Image Display Refnum"=refnum} ("output cluster"), "Image Display Refnum"=w323, "Current ROI Tool"=w333, "ROI Descriptor"=w326, "Shift"=w325, "Alt"=w324) -> (w328:T19)
                n163 = Bundle By Name(cluster=w334, "Phasor Plot Display Event"=w337) -> (w339:T7)
                n164 = Bundle By Name(cluster=T16 {"AlliGator Q Event"=enum."Phasor Plot:Mouse Up", "Data"=variant} ("AlliGator Actions out"), "Data"=w328) -> (w329:T16)
                n165 = Build Array(w329) -> (w327:T16[])
              }
            }
          }
        }
      }
      event Mouse Down {
        n166 = event-data() -> ("CtlRef"=w340:refnum<vi>)  [unwired: 1 in]
        n167 = Unbundle By Name(w343) -> ("Phasor Plote Display Range Event"=w344:refnum<event-registration>)
        n168 = register-events(reference=w344, refnum<vi> refnum ("event source"), w340, w340, w340) -> (reference out=w341:refnum<event-registration>, error out=w342:errorcluster)  [unwired: 1 in]
        n169 = Bundle By Name(cluster=w343, "Phasor Plote Display Range Event"=w341) -> ()  [unwired: 1 out]
      }
      event Mouse Leave; Mouse Up {
        w352 = refnum<vi> refnum ("event source")
        n170 = event-data() -> ("CtlRef"=w350:refnum<vi>)  [unwired: 1 in]
        n171 = Unbundle By Name(w349) -> ("Phasor Plote Display Range Event"=w351:refnum<event-registration>)
        n172 = register-events(reference=w351, w350, w352, w352, w352) -> (reference out=w346:refnum<event-registration>, error out=w347:errorcluster)  [unwired: 1 in]
        n173 = Bundle By Name(cluster=w349, "Phasor Plote Display Range Event"=w346) -> (w348:T7)
      }
      event Mouse Move {
        n174 = event-data() -> ("Time"=w355:u32)  [unwired: 1 in]
        n175 = case shown="True" w354 {
          tunnel: [_ w359] -> w353
          tunnel: w355 -> [_ w357]
          frame False {
          }
          frame True {
            w356 = T16 {"AlliGator Q Event"=enum."Phasor Plot:Display Range Mouse Move", "Data"=variant} ("Time-Gated Phasor Q Element")
            n176 = call "AlliGator Filter Event.vi"("Time"=w357, "AlliGatorr Q Element"=w356) -> ("Filter Event?"=w358:bool)  [unwired: 8 in, 1 out]
            n177 = case shown="False" w358 {
              tunnel: [w361 _] -> w359
              tunnel: w356 -> [w360 _]
              frame False {
                n178 = Build Array(w360) -> (w361:T16[])
              }
              frame True {
              }
            }
          }
        }
      }
    }
    n179 = call "AlliGator Settings Storage.vi"("AlliGator Settings List"=AlliGator_Settings_List."Miscellaneous:Verbose Error Mode") -> ("Variant Data out"=w66:variant)  [unwired: 9 in, 1 out]
    n180 = call-poly "Variant to Data.vi"("Variant"=w66) -> ("Value"=w59:bool)  [unwired: 8 in]
    n181 = call "Send Message to Notebook.vi"("Error In"=w61, "Text"=w58, "Notebook Queue"=w60) -> ("Error Out"=w63:errorcluster, "Notebook Queue"=w62:refnum<queue>)  [unwired: 5 in]
    n182 = call "Light Theme Message Style.vi"() -> ()  [unwired: 1 out]
    n183 = call "AlliGator Queue Non Empty Events.vi"("Actions"=w56, "AlliGator Q"=w57) -> ()  [unwired: 9 in, 1 out]
    n184 = call "Send Error to Notebook.vi"("error in (no error)"=w63, "Verbose Error Messages (T)"=w59, "State Machine Case Error Source"="Phasor Plot", "Notebook Q"=w62) -> ("Error Out"=w50:errorcluster)  [unwired: 7 in]
  }
  n185 = property on="Phasor Plot ROI Color" class="ColBox"("Val(Sgnl)"="Phasor Plot ROI Color") -> ()  [unwired: 2 in, 2 out]
  n186 = call "Tiny Clear Error.vi"("Error In"=w43) -> ("no Error Out"=w42:errorcluster)  [unwired: 8 in]
  n187 = Unregister For Events(event registration refnum=w44) -> (error out=w36:errorcluster)  [unwired: 1 in]
  n188 = invoke class="VI" method="FP.Close"(reference=w9, error in=w42) -> (error out=w37:errorcluster)  [unwired: 1 in, 2 out]
  n189 = Merge Errors(w37, w36) -> (w35:errorcluster)
  n190 = call "Tiny Clear Error.vi"("Error In"=w35) -> ()  [unwired: 8 in, 1 out]
